vi "libssh2_session_flag.vi"(8 "error in (no error)":errorcluster, 9 "value (0 = disabled)":i32, 10 "flag":T1, 11 "session":T2) -> (0 "error out":errorcluster)   [LabVIEW 2017, in "libssh2.lvlib"]
doc: "Set the value of a session flag."
uses:
  libssh2.lvlib
  Session Refnum.ctl
  libssh2_flag.ctl
  Not A Session.vi
  <vilib>/Utility/error.llb/Error Cluster From Error Code.vi
  Global Settings.vi
  Read Session Refnum.vi
  <vilib>/Utility/semaphor.llb/Acquire Semaphore.vi
  <vilib>/Utility/semaphor.llb/Release Semaphore.vi
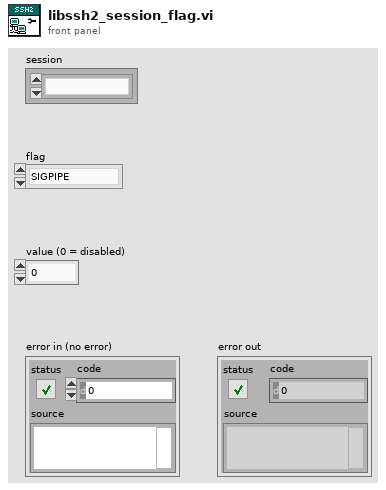
[diagram p1: front panel]
types:
  T1 = typedef "libssh2.lvlib/libssh2_flag.ctl" = enum16{"SIGPIPE", "COMPRESS", "QUOTE_PATHS"}
  T2 = typedef "libssh2.lvlib/Session Refnum.ctl" = refnum<k1>
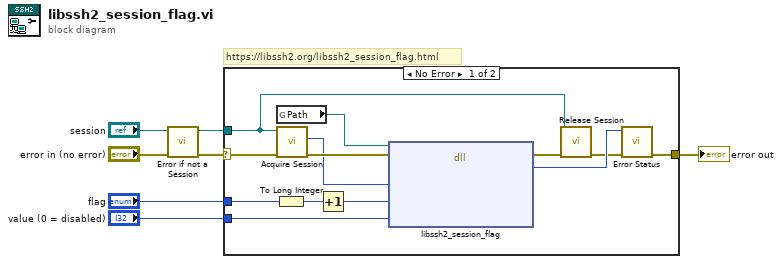
[diagram p0: block diagram]
diagram:
  # "https://libssh2.org/libssh2_session_flag.html"
  n1 = call "Error if not a Session.vi"("error in (no error)"="error in (no error)", "session"="session") -> ("error out"=w5:errorcluster, "session out"=w3:T2)  [unwired: 8 in]
  n2 = case shown="No Error" w5 {
    selector: w5 -> [w19 w21]
    tunnel: [w15 w21] -> w7
    tunnel: w3 -> [w8 _]
    tunnel: "flag" -> [w13 _]
    tunnel: "value (0 = disabled)" -> [w10 _]
    frame No Error {
      n3 = To Long Integer(number=w13) -> (32bit integer=w12:i32)
      n4 = global read "Global Settings.vi" "Path"() -> (w16:path)
      n5 = call "Acquire Session.vi"("error in (no error)"=w19, "session"=w8) -> ("error out"=w18:errorcluster, "LIBSSH2_SESSION*"=w17:u64)  [unwired: 7 in, 1 out]
      n6 = Increment(x=w12) -> (x+1=w11:i32)
      n7 = dll-call lib="?" fn="libssh2_session_flag"(path in=w16, error in=w18, "session"=w17, "flag"=w11, "value"=w10) -> (error out=w20:errorcluster, "return value"=w14:i32)  [unwired: 4 in, 1 out]
      n8 = call "Release Session.vi"("error in (no error)"=w20, "session"=w8) -> ("error out"=w9:errorcluster)  [unwired: 9 in]
      n9 = call "Error Status.vi"("error in (no error)"=w9, "return value"=w14) -> ("error out"=w15:errorcluster)  [unwired: 8 in, 1 out]
    }
    frame Error {
    }
  }
  "error out" <- w7
